vi "Init_Devices.vi"(8 "error in":errorcluster) -> (0 "error out":errorcluster, 2 "Error string":string)   [LabVIEW 2021]
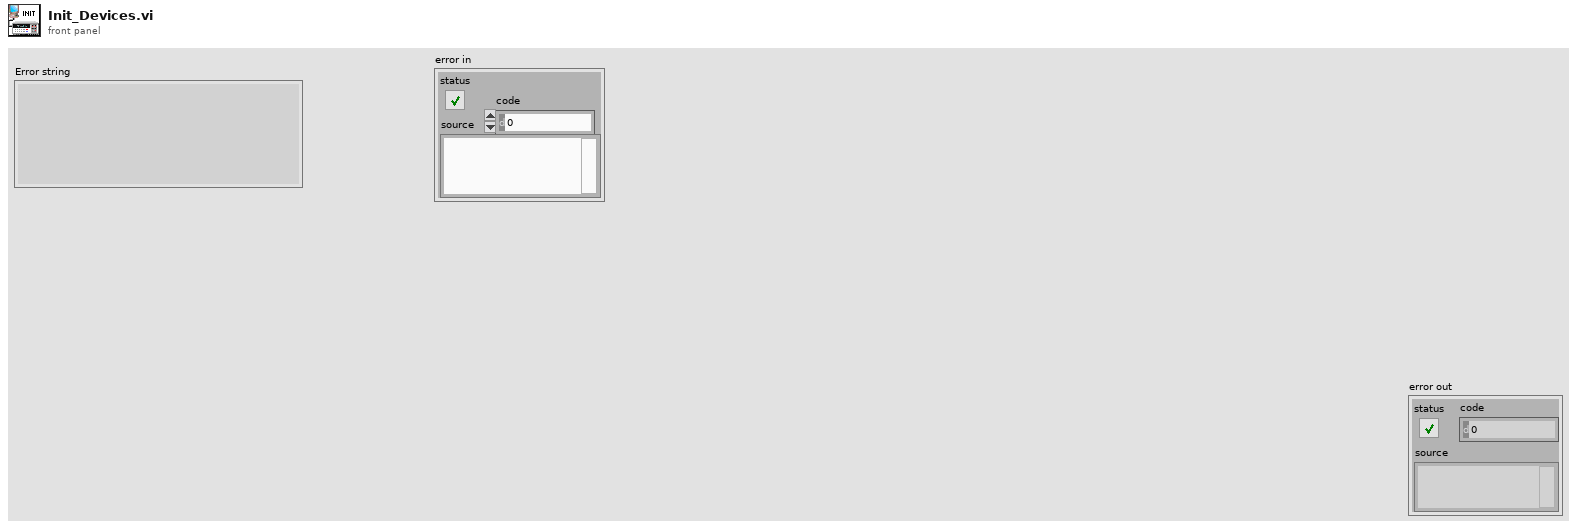
[diagram p1: front panel]
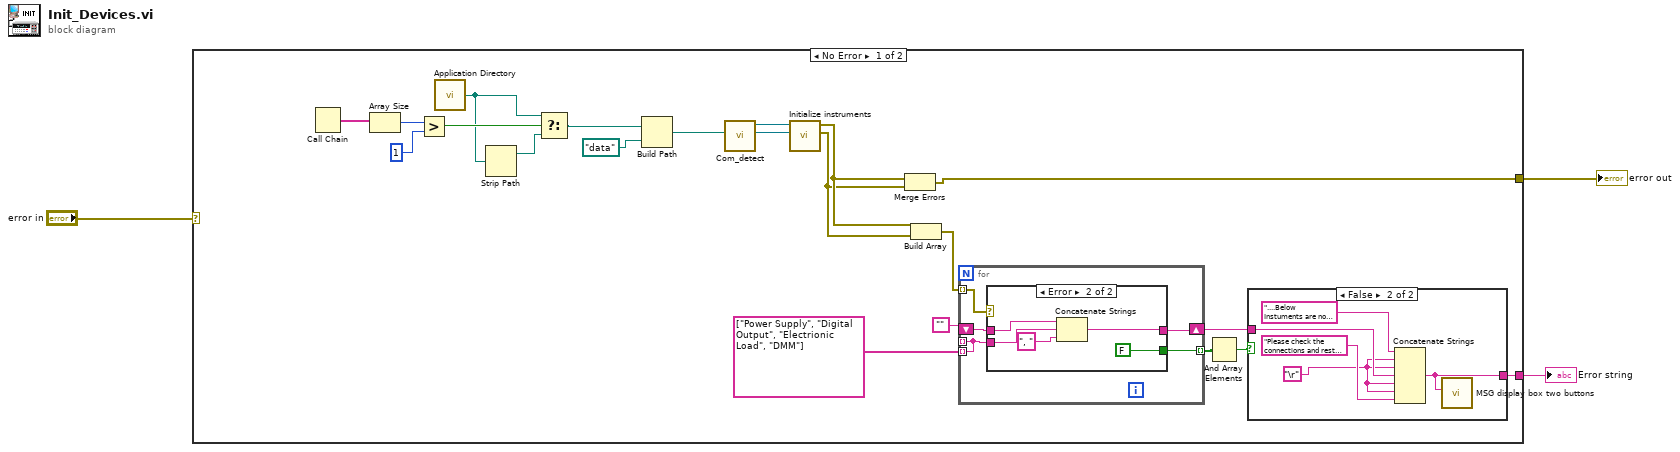
[diagram p0: block diagram]
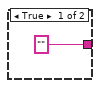
[diagram p2: hidden frame]
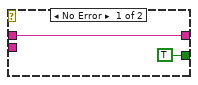
[diagram p3: hidden frame]
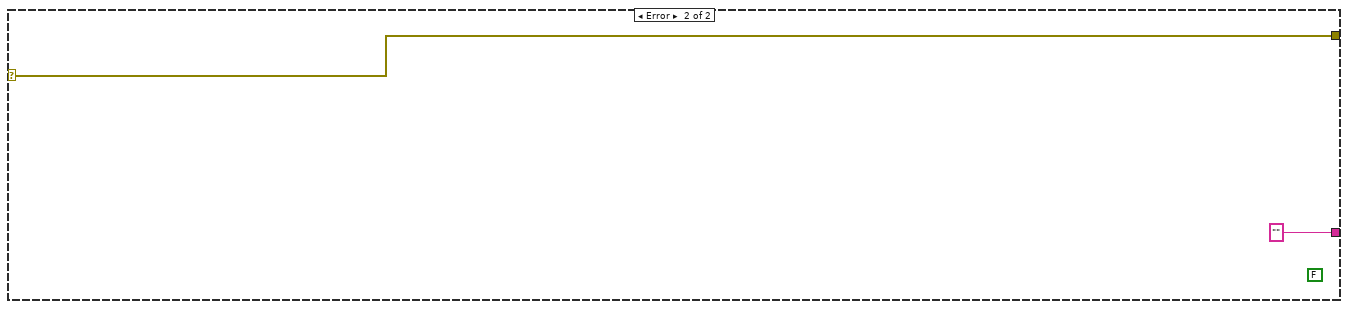
[diagram p4: hidden frame]
diagram:
  n1 = case shown="No Error" "error in" {
    selector: "error in" -> [_ w44]
    tunnel: [w17 w44] -> w1
    tunnel: [w22 ""] -> w2
    frame No Error {
      n2 = Call Chain() -> (call chain=w16:string[])
      n3 = Array Size(array=w16) -> (size(s)=w15:i32)
      n4 = Greater?(x=w15, y=1) -> (0:w13:bool)
      n5 = call <vilib>:"Application Directory.vi"() -> ("Application Directory"=w12:path)
      n6 = Strip Path(path=w12) -> (stripped path=w11:path)  [unwired: 1 out]
      n7 = Select(t=w12, s=w13, f=w11) -> (s? t:f=w9:path)
      n8 = Build Path(base path=w9, name or relative path=path "data") -> (appended path=w8:path)
      n9 = call "Com_detect.vi"("working directory"=w8) -> ("Barcode"=w4:refnum<visa-resource-name>, "HIPOT"=w7:refnum<visa-resource-name>)  [unwired: 8 in, 1 out]
      n10 = call "Initialize instruments.vi"("HIPOT"=w7, "Barcode"=w4) -> ("Power supply"=w6:errorcluster, "error out"=w5:errorcluster)  [unwired: 6 in]
      n11 = Merge Errors(w6, w5) -> (w17:errorcluster)
      n12 = Build Array(w6, w5) -> (w18:errorcluster[])
      n13 = for {
        tunnel: w18 -> [w31] mode=indexing
        tunnel: [w32] -> _ mode=indexing
        shift-right: [w34] -> w23
        shift-left: "" -> [w35]
        tunnel: [w33] -> w21 mode=indexing
        tunnel: string[] ["Power Supply", "Digital Output", "Electrionic Load", "DMM"] -> [w32] mode=indexing
        n14 = case shown="Error" w31 {
          tunnel: w32 -> [_ w41]
          tunnel: w35 -> [w37 w42]
          tunnel: [w37 w39] -> w34
          tunnel: [TRUE FALSE] -> w33
          frame No Error {
          }
          frame Error {
            n15 = Concatenate Strings(w42, w41, ", " ("string")) -> (w39:string)
          }
        }
      }
      n16 = And Array Elements(Boolean array=w21) -> (logical AND=w20:bool)
      n17 = case shown="False" w20 {
        tunnel: w23 -> [_ w30]
        tunnel: ["" w26] -> w22
        frame True {
        }
        frame False {
          w27 = "\r"
          n18 = Concatenate Strings("....Below Instuments are not properly initialised..." ("Initial Message"), w27, w27, w30, w27, w27, "Please check the connections and restart the application" ("Initial Message")) -> (w26:string)
          n19 = call "MSG display box two buttons.vi"("input string"=w26) -> ()  [unwired: 9 in, 2 out]
        }
      }
    }
    frame Error {
      (unwired) FALSE ("OK Button 2")
    }
  }
  "error out" <- w1
  "Error string" <- w2
